vi "GenerateDependencyList.vi"(8 "error in (no error)":errorcluster, 10 "Path to Check":path, 11 "CDependencyInspector in":refnum<class "CDependencyInspection.lvclass">) -> (0 "error out":errorcluster, 1 "Number of Files":i32, 3 "CDependencyInspector out":refnum<class "CDependencyInspection.lvclass">, 4 "Debug string":string)   [LabVIEW 2020, in "DependencyInspection.lvlib" / "CDependencyInspection.lvclass"]
uses:
  CDependencyInspection.lvclass
  CDependencyQueue/CDependencyQueue.lvclass
  CVisitedSet/CVisitedSet.lvclass
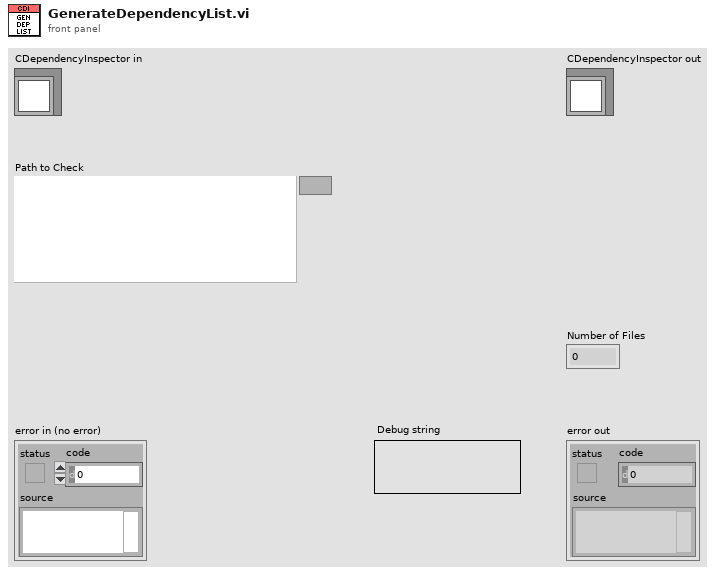
[diagram p1: front panel]
types:
  T1 = typedef "NI_FileType.lvlib/LVFileType.ctl" = enum32{"Invalid file", "Unknown type", "Instrument", "Control", "Polymorphic VI", "Project", "Library", "LVClass", "XControl", "XNode", "Shared library", ".NET assembly", "ActiveX interface", "CIN", "Run-time menu", "Palette menu", "Help file", "LLB", "XNode Edit Dependency", "Class Private Data Control", "Statechart", "MathScript .m file", "Ladder Diagram", "LVLibp", "XNode Build Dependency"}
  T2 = cluster{"path":path, "delimited name":string, "type":T1, "iState":u32, "iStyle":u16, "wStyle":u16, "buttons":u16, "viflags":u32, "viflags2":u32, "links":u32[]}[]
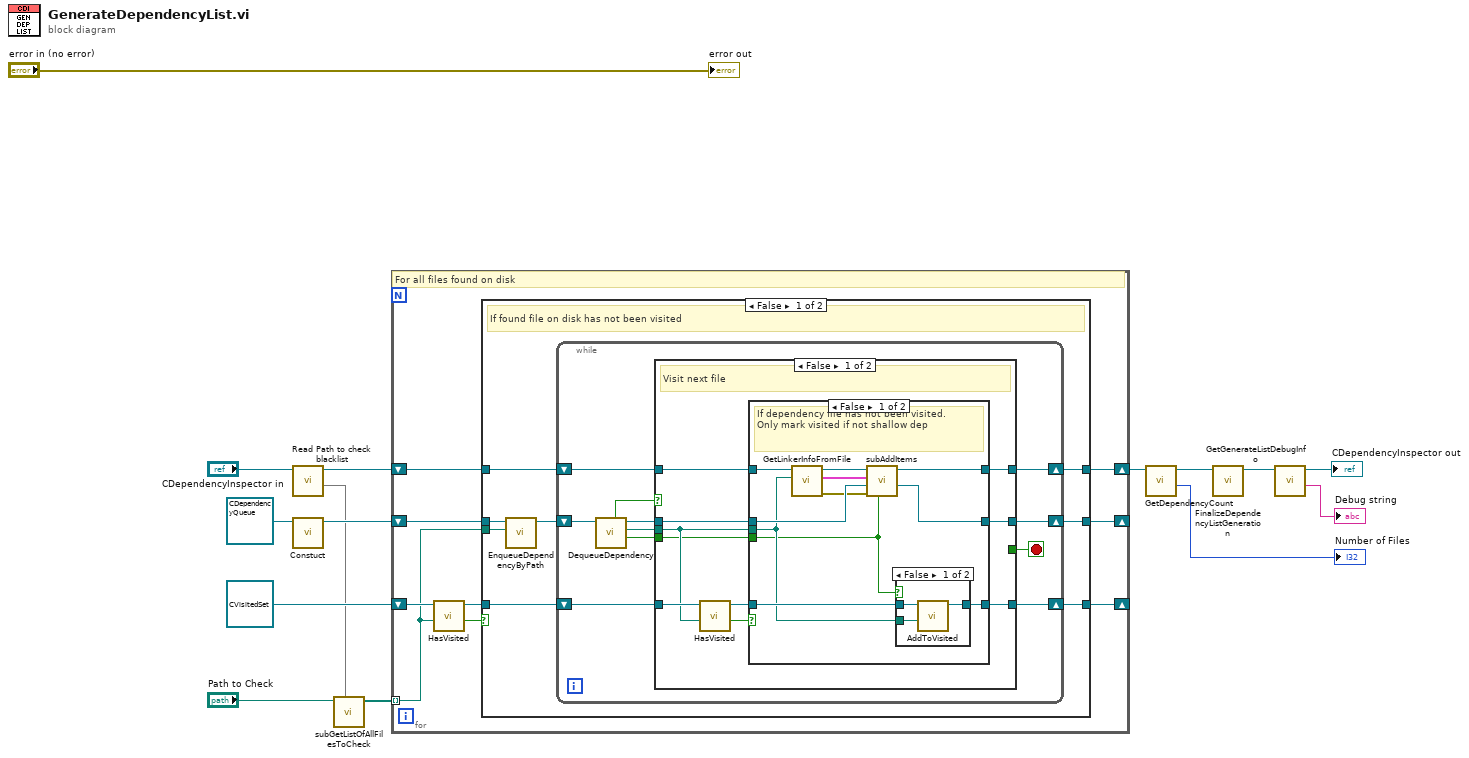
[diagram p0: block diagram]
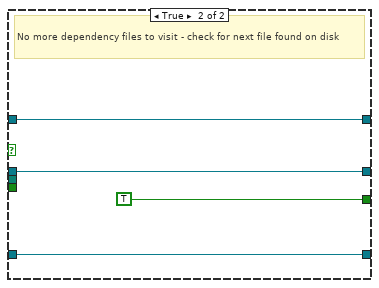
[diagram p4: hidden frame]
diagram:
  n1 = call-dynamic "Read Path to check blacklist.vi"("CDependencyInspection in"="CDependencyInspector in") -> ("Path to check blacklist"=w1:set{string}, "CDependencyInspection out"=w2:refnum<class "CDependencyInspection.lvclass">)  [unwired: 9 in]
  n2 = call-dynamic "Constuct.vi"("CDependencyQueue in"=refnum<class "CDependencyQueue.lvclass"> refnum ("DGML_Generator_Helper.lvlib:CDependencyQueue.lvclass")) -> ("CDependencyQueue out"=w12:refnum<class "CDependencyQueue.lvclass">)  [unwired: 9 in, 1 out]
  n3 = call "subGetListOfAllFilesToCheck.vi"("Path to check blacklist"=w1, "Path to Check"="Path to Check") -> ("All Files in Dir"=w14:path[])  [unwired: 9 in]
  n4 = for {
    tunnel: w14 -> [w16] mode=indexing
    shift-right: [w19] -> w8
    shift-left: w2 -> [w24]
    shift-right: [w18] -> _
    shift-left: w12 -> [w23]
    shift-right: [w20] -> _
    shift-left: refnum<class "CVisitedSet.lvclass"> refnum ("DGML_Generator_Helper.lvlib:CVisitedSet.lvclass") -> [w22]
    # "For all files found on disk"
    n5 = call-dynamic "HasVisited.vi"("Path"=w16, "CVisitedSet in"=w22) -> ("found?"=w17:bool, "CVisitedSet out"=w21:refnum<class "CVisitedSet.lvclass">)  [unwired: 7 in, 1 out]
    n6 = case shown="False" w17 {
      tunnel: w24 -> [w32 w78]
      tunnel: w23 -> [w27 w77]
      tunnel: w21 -> [w31 w76]
      tunnel: [w30 w76] -> w20
      tunnel: [w29 w78] -> w19
      tunnel: [w28 w77] -> w18
      tunnel: w16 -> [w25 _]
      frame False {
        # "If found file on disk has not been visited"
        n7 = call-dynamic "EnqueueDependencyByPath.vi"("Path"=w25, "CDependencyQueue in"=w27) -> ("CDependencyQueue out"=w26:refnum<class "CDependencyQueue.lvclass">)  [unwired: 8 in, 1 out]
        n8 = while {
          shift-right: [w40] -> w29
          shift-left: w32 -> [w43]
          shift-right: [w39] -> w28
          shift-left: w26 -> [w38]
          shift-right: [w41] -> w30
          shift-left: w31 -> [w42]
          stop <- w34 stop-if-true
          n9 = call-dynamic "DequeueDependency.vi"("CDependencyQueue in"=w38) -> ("Shallow deps?"=w33:bool, "Path"=w36:path, "CDependencyQueue out"=w37:refnum<class "CDependencyQueue.lvclass">, "timed out?"=w35:bool)  [unwired: 6 in, 1 out]
          n10 = case shown="False" w35 {
            tunnel: w43 -> [w53 w75]
            tunnel: w37 -> [w52 w74]
            tunnel: w42 -> [w51 w73]
            tunnel: [w49 w73] -> w41
            tunnel: [w48 w75] -> w40
            tunnel: [w47 w74] -> w39
            tunnel: w36 -> [w46 _]
            tunnel: [_ TRUE] -> w34
            tunnel: w33 -> [w44 _]
            frame False {
              # "Visit next file"
              n11 = call-dynamic "HasVisited.vi"("Path"=w46, "CVisitedSet in"=w51) -> ("found?"=w45:bool, "CVisitedSet out"=w50:refnum<class "CVisitedSet.lvclass">)  [unwired: 7 in, 1 out]
              n12 = case shown="False" w45 {
                tunnel: w53 -> [w60 w71]
                tunnel: w52 -> [w64 w70]
                tunnel: w50 -> [w63 w69]
                tunnel: [w62 w69] -> w49
                tunnel: [w54 w71] -> w48
                tunnel: [w61 w70] -> w47
                tunnel: w46 -> [w59 _]
                tunnel: w44 -> [w55 _]
                frame False {
                  # "If dependency file has not been visited.\nOnly mark visited if not shallow dep"
                  n13 = call "GetLinkerInfoFromFile.vi"("path in"=w59, "CDependencyInspector in"=w60) -> ("error out"=w57:errorcluster, "Linker.Read Info From File"=w58:T2, "CDependencyInspector out"=w56:refnum<class "CDependencyInspection.lvclass">)  [unwired: 7 in]
                  n14 = call "subAddItems.vi"("Shallow deps?"=w55, "error in (no error)"=w57, "CDependencyQueue in"=w64, "Linker.Read Info From File"=w58, "CDependencyInspector in"=w56) -> ("CDependencyQueue out"=w61:refnum<class "CDependencyQueue.lvclass">, "CDependencyInspector out"=w54:refnum<class "CDependencyInspection.lvclass">)  [unwired: 4 in, 1 out]
                  n15 = case shown="False" w55 {
                    tunnel: w63 -> [w67 w68]
                    tunnel: [w66 w68] -> w62
                    tunnel: w59 -> [w65 _]
                    frame False {
                      n16 = call-dynamic "AddToVisited.vi"("Path"=w65, "CVisitedSet in"=w67) -> ("CVisitedSet out"=w66:refnum<class "CVisitedSet.lvclass">)  [unwired: 8 in, 1 out]
                    }
                    frame True {
                    }
                  }
                }
                frame True {
                  # "Seen this file before"
                }
              }
            }
            frame True {
              # "No more dependency files to visit - check for next file found on disk"
            }
          }
        }
      }
      frame True {
        # "Seen this file before"
      }
    }
  }
  n17 = call-dynamic "GetDependencyCount.vi"("CDependencyInspector in"=w8) -> ("Count"=→"Number of Files":i32, "CDependencyInspector out"=w6:refnum<class "CDependencyInspection.lvclass">)  [unwired: 8 in, 1 out]
  n18 = call-dynamic "FinalizeDependencyListGeneration.vi"("CDependencyInspector in"=w6) -> ("CDependencyInspector out"=w5:refnum<class "CDependencyInspection.lvclass">)  [unwired: 9 in, 1 out]
  n19 = call-dynamic "GetGenerateListDebugInfo.vi"("CDependencyInspector in"=w5) -> ("Debug string"=→"Debug string":string, "CDependencyInspector out"=→"CDependencyInspector out":refnum<class "CDependencyInspection.lvclass">)  [unwired: 8 in, 1 out]
  "error out" <- "error in (no error)"
